vi "Set Filter Path.vi"(8 "error in (no error)":errorcluster caption="에러 입력(에러 없음)", 10 "Filter path":T1, 11 "Instrument Manager 입력":refnum<class "Instrument Manager.lvclass">) -> (0 "error out":errorcluster caption="에러 출력", 3 "Instrument Manager 출력":refnum<class "Instrument Manager.lvclass">)   [LabVIEW 2023, in "Instrument Manager.lvclass"]
uses:
  Instrument Manager.lvclass
  Module/CE RF Switch Box/Type Definition/Filter path.ctl
  Instrument Manager.lvclass/Instrument Manager.ctl
  Module/CE RF Switch Box/RF Filter Box/RF Filter Box.lvclass
  Module/CE RF Switch Box/RF Switch Box.lvlib
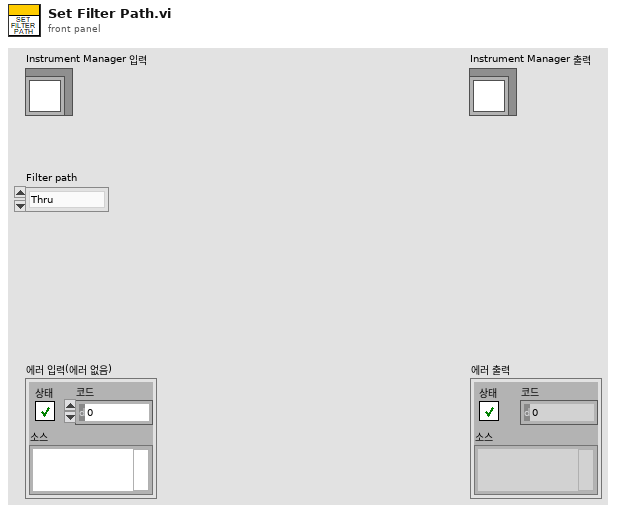
[diagram p1: front panel]
types:
  T1 = typedef "RF Switch Box.lvlib/Filter path.ctl" = enum16{"Thru", "Direct Amp", "1G HPF", "3G HPF", "7G HPF", "6G HPF", "port 1", "port 2", "port 3", "port 4", "port 5", "port 6", "port 7", "port 8", "port 9", "port 10", "port 11", "port 12", "port 13", "port 14", "port 15", "port 16", "port 17", "port 18"}
  T2 = cluster{"Anritsu Call Box":refnum<class "Anritsu Call Box.lvclass">, "Spectrum Analyzer":refnum<class "Interface_Spectrum.lvclass">, "RF Switch Box":refnum<class "RF Filter Box.lvclass">, "Turn Table":refnum<class "Interface - Turn Table.lvclass">, "Mast":refnum<class "Interface - Mast.lvclass">, "3D Controller":refnum<class "Interface_3D Controller.lvclass">}
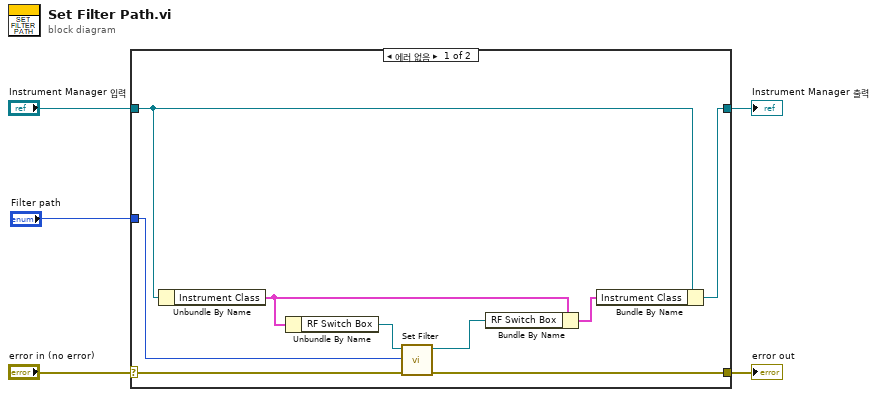
[diagram p0: block diagram]
diagram:
  n1 = case shown="에러 없음" "error in (no error)" {
    selector: "error in (no error)" -> [w13 w16]
    tunnel: [w11 w16] -> w4
    tunnel: [w7 w15] -> w2
    tunnel: "Instrument Manager 입력" -> [w8 w15]
    tunnel: "Filter path" -> [w12 _]
    frame No Error {
      n2 = Unbundle By Name(w8) -> ("Instrument Class"=w9:T2)
      n3 = Unbundle By Name(w9) -> ("RF Switch Box"=w14:refnum<class "RF Filter Box.lvclass">)
      n4 = call-dynamic "Set Filter.vi"("error in (no error)"=w13, "Filter path"=w12, "RF Filter Box 입력"=w14) -> ("error out"=w11:errorcluster, "RF Filter Box 출력"=w10:refnum<class "RF Filter Box.lvclass">)  [unwired: 7 in]
      n5 = Bundle By Name(cluster=w9, "RF Switch Box"=w10) -> (w6:T2)
      n6 = Bundle By Name(cluster=w8, "Instrument Class"=w6) -> (w7:refnum<class "Instrument Manager.lvclass">)
    }
    frame Error {
    }
  }
  "error out" <- w4
  "Instrument Manager 출력" <- w2
